vi "EQ.vi"(8 "error in (no error)":errorcluster, 10 "Audio Block In":dbl[][](array[numeric]), 11 "Channel in":refnum<class "Channel.lvclass">) -> (0 "error out":errorcluster, 2 "Audio Block Out":dbl[][](array[numeric]))   [LabVIEW 2019, in "Channel.lvclass"]
doc: "Perform 3-band (low, mid, high) equalization of the audio data using Butterworth filters."
uses:
  Channel.lvclass
  Channel.lvclass/Channel.ctl
  <vilib>/Analysis/3filter.llb/Filter Passband Type.ctl
  Packed Libraries/Globals.lvlibp/Constants.vi
  <vilib>/Analysis/3filter.llb/Butterworth Filter (DBL).vi
  <vilib>/Analysis/NI_AALBase.lvlib
  Packed Libraries/Globals.lvlibp
  Libraries/User Interface/User Interface.lvlib
  Packed Libraries/Audio Processing.lvlibp
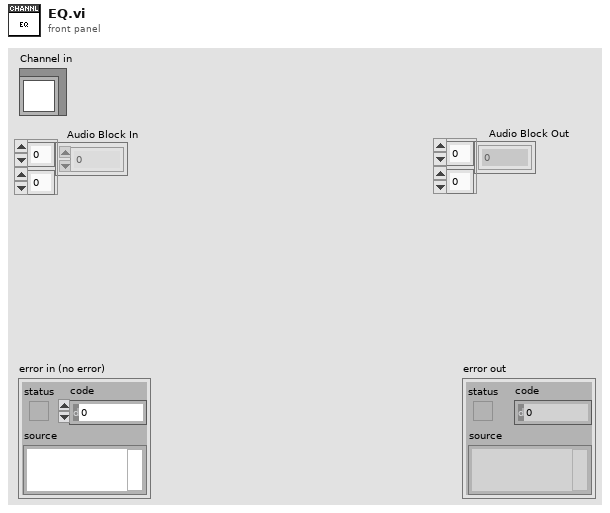
[diagram p1: front panel]
types:
  T1 = typedef "NI_AALBase.lvlib/Filter Passband Type.ctl" = enum32{"Lowpass", "Highpass", "Bandpass", "Bandstop"}
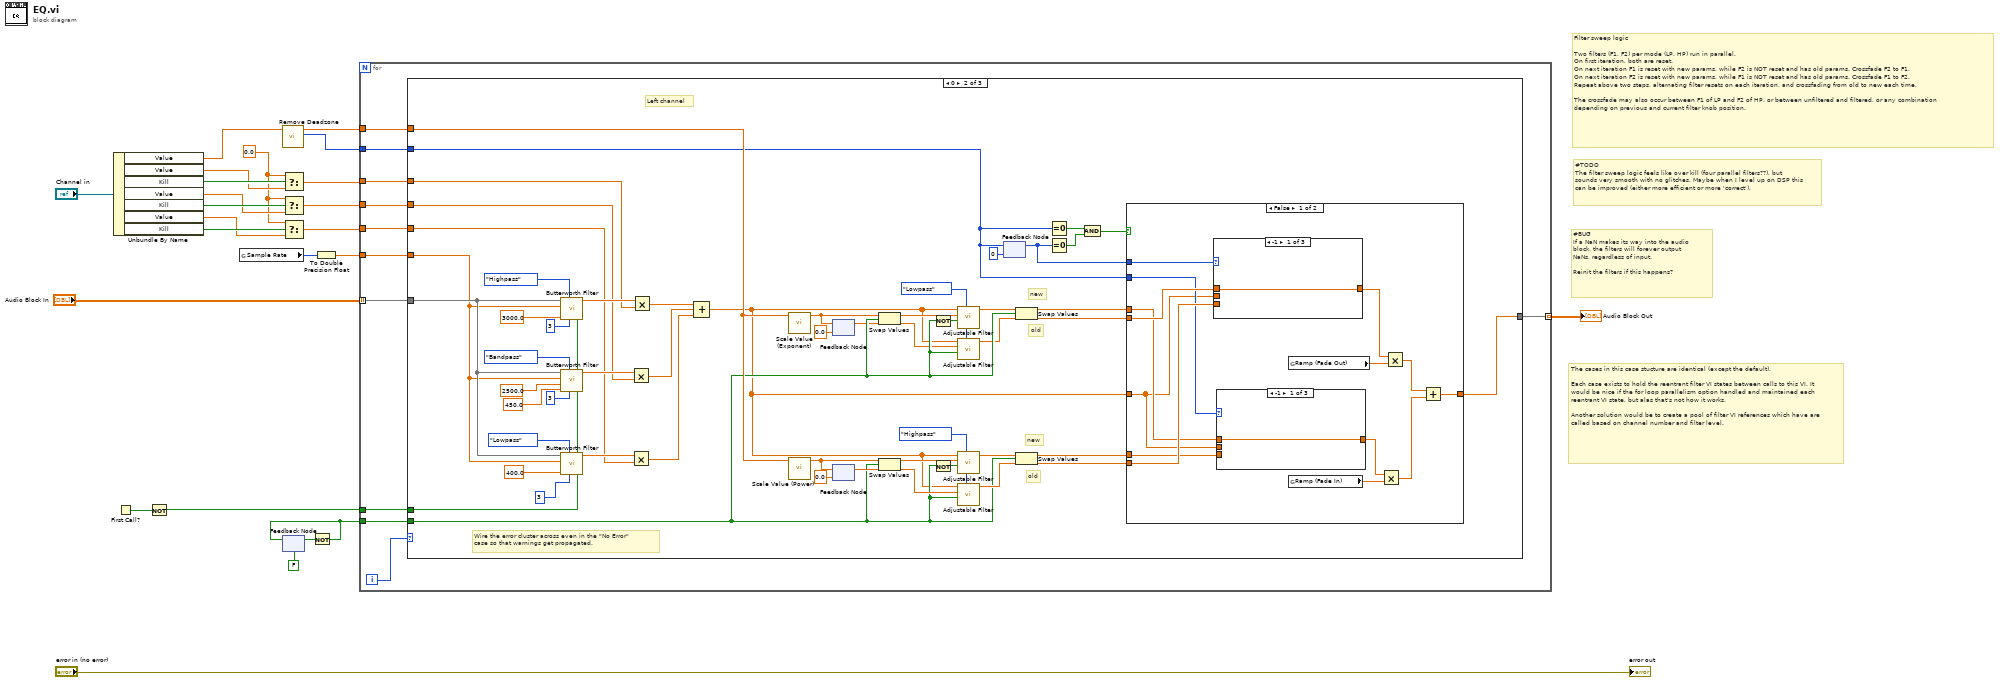
[diagram p0: block diagram]
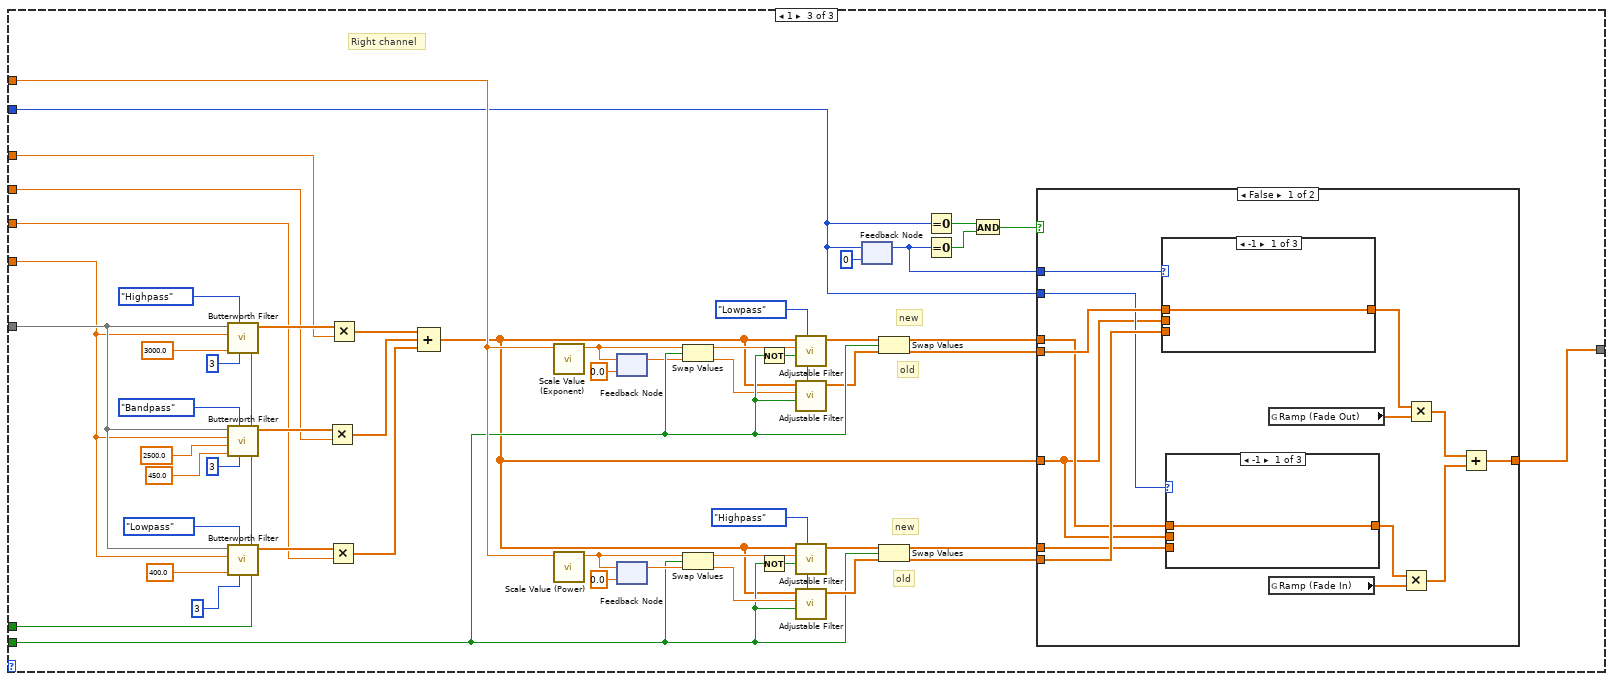
[diagram p8: hidden frame]
diagram:
  w17 = 0.0 ("t")
  # "Filter sweep logic\n\nTwo filters (F1, F2) per mode (LP, HP) run in parallel.\nOn first iteration, both are reset.\nOn next iteration F1 is reset with new params, while F2 is NOT reset and has old params. Crossfade F2 to F1.\nOn next iteration F2 is reset with new params, while F1 is NOT reset and has old params. Crossfade F1 to F2.\nRepeat above two steps, alternating filter resets on each iteration, and crossfading from old to new each time.\n\nThe crossfade may also occur between F1 of LP and F2 of HP, or between unfiltered and filtered, or any combination depending on previous and current filter knob position."
  # "#TODO\nThe filter sweep logic feels like over kill (four parallel filters??), but sounds very smooth with no glitches. Maybe when I level up on DSP this can be improved (either more efficient or more 'correct')."
  # "#BUG\nIf a NaN makes its way into the audio block, the filters will forever output NaNs, regardless of input.\n\nReinit the filters if this happens?"
  # "Wire the error cluster across even in the \"No Error\"\ncase so that warnings get propagated."
  # "The cases in this case stucture are identical (except the default).\n\nEach case exists to hold the reentrant filter VI states between calls to this VI. It would be nice if the for loop parallelism option handled and maintained each reentrant VI state, but alas that's not how it works.\n\nAnother solution would be to create a pool of filter VI references which have are called based on channel number and filter level."
  n1 = Unbundle By Name("Channel in") -> ("Value"=w6:dbl, "Value"=w20:dbl, "Kill"=w21:bool, "Value"=w18:dbl, "Kill"=w19:bool, "Value"=w15:dbl, "Kill"=w16:bool)
  n2 = First Call?() -> (First Call?: T/F=w11:bool)
  n3 = Not(x=w11) -> (.not. x?=w10:bool)
  n4 = global read "Constants.vi" "Sample Rate"() -> (w9:i32)
  n5 = call "Remove Deadzone.vi"("Value"=w6) -> ("Sign"=w4:i32, "Abs Value"=w5:dbl)  [unwired: 9 in]
  n6 = Select(t=w17, s=w21, f=w20) -> (s? t:f=w14:dbl)
  n7 = Select(t=w17, s=w19, f=w18) -> (s? t:f=w13:dbl)
  n8 = Select(t=w17, s=w16, f=w15) -> (s? t:f=w12:dbl)
  n9 = feedback #1(FALSE) -> (w2:bool)
  n10 = Not(x=w2) -> (.not. x?=w1:bool)
  n11 = feedback-in #1(w1) -> ()
  n12 = To Double Precision Float(number=w9) -> (double precision float=w8:dbl)
  n13 = for {
    tunnel: "Audio Block In" -> [w35] mode=indexing
    tunnel: w12 -> [w34]
    tunnel: w13 -> [w33]
    tunnel: w14 -> [w32]
    tunnel: [w26] -> w7 mode=indexing
    tunnel: w10 -> [w31]
    tunnel: w8 -> [w29]
    tunnel: w5 -> [w28]
    tunnel: w4 -> [w27]
    tunnel: w1 -> [w25]
    i -> [w30]
    n14 = case shown="0" w30 {
      tunnel: w35 -> [w36 w79 w154]
      tunnel: w34 -> [_ w78 w153]
      tunnel: w33 -> [_ w77 w152]
      tunnel: w32 -> [_ w76 w151]
      tunnel: [w36 w46 w121] -> w26
      tunnel: w31 -> [_ w75 w150]
      tunnel: w29 -> [_ w69 w144]
      tunnel: w28 -> [_ w60 w135]
      tunnel: w27 -> [_ w44 w119]
      tunnel: w25 -> [_ w59 w134]
      frame Default {
        # "Not expecting more than two channels, so pass them through unfiltered"
      }
      frame 0 {
        w51 = Filter_Passband_Type."Lowpass" ("Type (LP)")
        w61 = Filter_Passband_Type."Highpass" ("Type (LP)")
        # "old"
        # "new"
        # "old"
        # "new"
        # "Left channel"
        n15 = call-poly <vilib>:"Butterworth Filter.vi"("init/cont (init:F)"=w75, "order"=3, "filter type"=Filter_Passband_Type."Highpass", "low cutoff freq: fl"=3000.0 ("high cutoff freq: fh"), "sampling freq: fs"=w69, "X"=w79) -> ("Filtered X"=w85:dbl[])  [unwired: 2 in, 1 out]
        n16 = call-poly <vilib>:"Butterworth Filter.vi"("init/cont (init:F)"=w75, "order"=3, "filter type"=Filter_Passband_Type."Bandpass", "low cutoff freq: fl"=450.0, "high cutoff freq: fh"=2500.0, "sampling freq: fs"=w69, "X"=w79) -> ("Filtered X"=w84:dbl[])  [unwired: 1 in, 1 out]
        n17 = call-poly <vilib>:"Butterworth Filter.vi"("init/cont (init:F)"=w75, "order"=3, "filter type"=Filter_Passband_Type."Lowpass", "low cutoff freq: fl"=400.0, "sampling freq: fs"=w69, "X"=w79) -> ("Filtered X"=w82:dbl[])  [unwired: 2 in, 1 out]
        n18 = Multiply(x=w84, y=w77) -> (x*y=w83:dbl[])
        n19 = Multiply(x=w82, y=w78) -> (x*y=w70:dbl[])
        n20 = Multiply(x=w85, y=w76) -> (x*y=w71:dbl[])
        n21 = Compound Arithmetic op=ADD(w71, w83, w70) -> (w47:dbl[])
        n22 = call "Scale Value (Exponent).vi"("Value"=w60) -> ("Scaled Value"=w57:dbl)  [unwired: 10 in]
        n23 = call "Scale Value (Power).vi"("Value"=w60) -> ("Scaled Value"=w67:dbl)  [unwired: 10 in]
        n24 = feedback #2(0.0 ("Scaled Value")) -> (w58:dbl)
        n25 = feedback-in #2(w57) -> ()
        n26 = feedback #3(0.0 ("Scaled Value")) -> (w68:dbl)
        n27 = feedback-in #3(w67) -> ()
        n28 = Swap Values(12:w57, 13:w59, 14:w58) -> (1:w56:dbl, 3:w55:dbl)
        n29 = Swap Values(12:w67, 13:w59, 14:w68) -> (1:w66:dbl, 3:w65:dbl)
        n30 = Not(x=w59) -> (.not. x?=w54:bool)
        n31 = Not(x=w59) -> (.not. x?=w64:bool)
        n32 = call "Adjustable Filter.vi"("Filter Type"=w51, "Reset Filter"=w54, "Frequency"=w56, "Audio Data"=w47) -> ("Filtered Audio Data"=w53:dbl[])  [unwired: 7 in]
        n33 = call "Adjustable Filter.vi"("Filter Type"=w51, "Reset Filter"=w59, "Frequency"=w55, "Audio Data"=w47) -> ("Filtered Audio Data"=w52:dbl[])  [unwired: 7 in]
        n34 = call "Adjustable Filter.vi"("Filter Type"=w61, "Reset Filter"=w64, "Frequency"=w66, "Audio Data"=w47) -> ("Filtered Audio Data"=w63:dbl[])  [unwired: 7 in]
        n35 = call "Adjustable Filter.vi"("Filter Type"=w61, "Reset Filter"=w59, "Frequency"=w65, "Audio Data"=w47) -> ("Filtered Audio Data"=w62:dbl[])  [unwired: 7 in]
        n36 = feedback #4(0 ("Sign")) -> (w45:i32)
        n37 = feedback-in #4(w44) -> ()
        n38 = Swap Values(12:w53, 13:w59, 14:w52) -> (1:w43:dbl[], 3:w42:dbl[])
        n39 = Swap Values(12:w63, 13:w59, 14:w62) -> (1:w41:dbl[], 3:w40:dbl[])
        n40 = Equal To 0?(x=w44) -> (x = 0?=w50:bool)
        n41 = Equal To 0?(x=w45) -> (x = 0?=w49:bool)
        n42 = And(x=w50, y=w49) -> (x .and. y?=w48:bool)
        n43 = case shown="False" w48 {
          tunnel: w47 -> [w97 w111]
          tunnel: [w91 w111] -> w46
          tunnel: w45 -> [w104 _]
          tunnel: w44 -> [w99 _]
          tunnel: w43 -> [w98 _]
          tunnel: w42 -> [w103 _]
          tunnel: w41 -> [w96 _]
          tunnel: w40 -> [w102 _]
          frame False {
            n44 = case shown="-1" w104 {
              tunnel: w103 -> [w108 _ _]
              tunnel: w97 -> [_ w109 _]
              tunnel: w102 -> [_ _ w110]
              tunnel: [w108 w109 w110] -> w100
              frame -1 {
              }
              frame 0, Default {
              }
              frame 1 {
              }
            }
            n45 = case shown="-1" w99 {
              tunnel: w98 -> [w105 _ _]
              tunnel: w97 -> [_ w106 _]
              tunnel: w96 -> [_ _ w107]
              tunnel: [w105 w106 w107] -> w94
              frame -1 {
              }
              frame 0, Default {
              }
              frame 1 {
              }
            }
            n46 = global read "Constants.vi" "Ramp (Fade Out)"() -> (w101:dbl[])
            n47 = global read "Constants.vi" "Ramp (Fade In)"() -> (w95:dbl[])
            n48 = Multiply(x=w94, y=w95) -> (x*y=w92:dbl[])
            n49 = Multiply(x=w100, y=w101) -> (x*y=w93:dbl[])
            n50 = Add(x=w93, y=w92) -> (x+y=w91:dbl[])
          }
          frame True {
          }
        }
      }
      frame 1 {
        w126 = Filter_Passband_Type."Lowpass" ("Type (LP)")
        w136 = Filter_Passband_Type."Highpass" ("Type (LP)")
        # "old"
        # "new"
        # "old"
        # "new"
        # "Right channel"
        n51 = call-poly <vilib>:"Butterworth Filter.vi"("init/cont (init:F)"=w150, "order"=3, "filter type"=Filter_Passband_Type."Highpass", "low cutoff freq: fl"=3000.0 ("high cutoff freq: fh"), "sampling freq: fs"=w144, "X"=w154) -> ("Filtered X"=w160:dbl[])  [unwired: 2 in, 1 out]
        n52 = call-poly <vilib>:"Butterworth Filter.vi"("init/cont (init:F)"=w150, "order"=3, "filter type"=Filter_Passband_Type."Bandpass", "low cutoff freq: fl"=450.0, "high cutoff freq: fh"=2500.0, "sampling freq: fs"=w144, "X"=w154) -> ("Filtered X"=w159:dbl[])  [unwired: 1 in, 1 out]
        n53 = call-poly <vilib>:"Butterworth Filter.vi"("init/cont (init:F)"=w150, "order"=3, "filter type"=Filter_Passband_Type."Lowpass", "low cutoff freq: fl"=400.0, "sampling freq: fs"=w144, "X"=w154) -> ("Filtered X"=w157:dbl[])  [unwired: 2 in, 1 out]
        n54 = Multiply(x=w159, y=w152) -> (x*y=w158:dbl[])
        n55 = Multiply(x=w157, y=w153) -> (x*y=w145:dbl[])
        n56 = Multiply(x=w160, y=w151) -> (x*y=w146:dbl[])
        n57 = Compound Arithmetic op=ADD(w146, w158, w145) -> (w122:dbl[])
        n58 = call "Scale Value (Exponent).vi"("Value"=w135) -> ("Scaled Value"=w132:dbl)  [unwired: 10 in]
        n59 = call "Scale Value (Power).vi"("Value"=w135) -> ("Scaled Value"=w142:dbl)  [unwired: 10 in]
        n60 = feedback #5(0.0 ("Scaled Value")) -> (w133:dbl)
        n61 = feedback-in #5(w132) -> ()
        n62 = feedback #6(0.0 ("Scaled Value")) -> (w143:dbl)
        n63 = feedback-in #6(w142) -> ()
        n64 = Swap Values(12:w132, 13:w134, 14:w133) -> (1:w131:dbl, 3:w130:dbl)
        n65 = Swap Values(12:w142, 13:w134, 14:w143) -> (1:w141:dbl, 3:w140:dbl)
        n66 = Not(x=w134) -> (.not. x?=w129:bool)
        n67 = Not(x=w134) -> (.not. x?=w139:bool)
        n68 = call "Adjustable Filter.vi"("Filter Type"=w126, "Reset Filter"=w129, "Frequency"=w131, "Audio Data"=w122) -> ("Filtered Audio Data"=w128:dbl[])  [unwired: 7 in]
        n69 = call "Adjustable Filter.vi"("Filter Type"=w126, "Reset Filter"=w134, "Frequency"=w130, "Audio Data"=w122) -> ("Filtered Audio Data"=w127:dbl[])  [unwired: 7 in]
        n70 = call "Adjustable Filter.vi"("Filter Type"=w136, "Reset Filter"=w139, "Frequency"=w141, "Audio Data"=w122) -> ("Filtered Audio Data"=w138:dbl[])  [unwired: 7 in]
        n71 = call "Adjustable Filter.vi"("Filter Type"=w136, "Reset Filter"=w134, "Frequency"=w140, "Audio Data"=w122) -> ("Filtered Audio Data"=w137:dbl[])  [unwired: 7 in]
        n72 = feedback #7(0 ("Sign")) -> (w120:i32)
        n73 = feedback-in #7(w119) -> ()
        n74 = Swap Values(12:w128, 13:w134, 14:w127) -> (1:w118:dbl[], 3:w117:dbl[])
        n75 = Swap Values(12:w138, 13:w134, 14:w137) -> (1:w116:dbl[], 3:w115:dbl[])
        n76 = Equal To 0?(x=w119) -> (x = 0?=w125:bool)
        n77 = Equal To 0?(x=w120) -> (x = 0?=w124:bool)
        n78 = And(x=w125, y=w124) -> (x .and. y?=w123:bool)
        n79 = case shown="False" w123 {
          tunnel: w122 -> [w172 w186]
          tunnel: [w166 w186] -> w121
          tunnel: w120 -> [w179 _]
          tunnel: w119 -> [w174 _]
          tunnel: w118 -> [w173 _]
          tunnel: w117 -> [w178 _]
          tunnel: w116 -> [w171 _]
          tunnel: w115 -> [w177 _]
          frame False {
            n80 = case shown="-1" w179 {
              tunnel: w178 -> [w183 _ _]
              tunnel: w172 -> [_ w184 _]
              tunnel: w177 -> [_ _ w185]
              tunnel: [w183 w184 w185] -> w175
              frame -1 {
              }
              frame 0, Default {
              }
              frame 1 {
              }
            }
            n81 = case shown="-1" w174 {
              tunnel: w173 -> [w180 _ _]
              tunnel: w172 -> [_ w181 _]
              tunnel: w171 -> [_ _ w182]
              tunnel: [w180 w181 w182] -> w169
              frame -1 {
              }
              frame 0, Default {
              }
              frame 1 {
              }
            }
            n82 = global read "Constants.vi" "Ramp (Fade Out)"() -> (w176:dbl[])
            n83 = global read "Constants.vi" "Ramp (Fade In)"() -> (w170:dbl[])
            n84 = Multiply(x=w169, y=w170) -> (x*y=w167:dbl[])
            n85 = Multiply(x=w175, y=w176) -> (x*y=w168:dbl[])
            n86 = Add(x=w168, y=w167) -> (x+y=w166:dbl[])
          }
          frame True {
          }
        }
      }
    }
  }
  "Audio Block Out" <- w7
  "error out" <- "error in (no error)"
